vi "Read_Time_array_formation_VI.vi"(0 "Right Read MAX":string, 5 "読み取り配列":string, 9 "リード方向総合":enum16{"5’→3'", "3'→5'"}(ring), 11 "配列開始番号":i32, 12 "配列終了番号":i32) -> (1 "読み取り開始番号":i32, 3 "読み取り終了番号":i32, 4 "Base Number":i32[](array[numeric]), 6 "核酸塩基配列開始番号":i32, 10 "核酸塩基配列終了番号":i32, 13 "RRead N":i32[](array[numeric]), 14 "RR(%)":dbl, 15 "配列情報":bool[](array[boolean]))   [LabVIEW 2018]
panel:
  out "長さ 2":i32
  out "長さ":i32
  out "前":i32
  out "中心":i32
  out "後":i32
  out "部分文字列の後":string
  out "一致部分文字列":string
  out "部分文字列の前":string
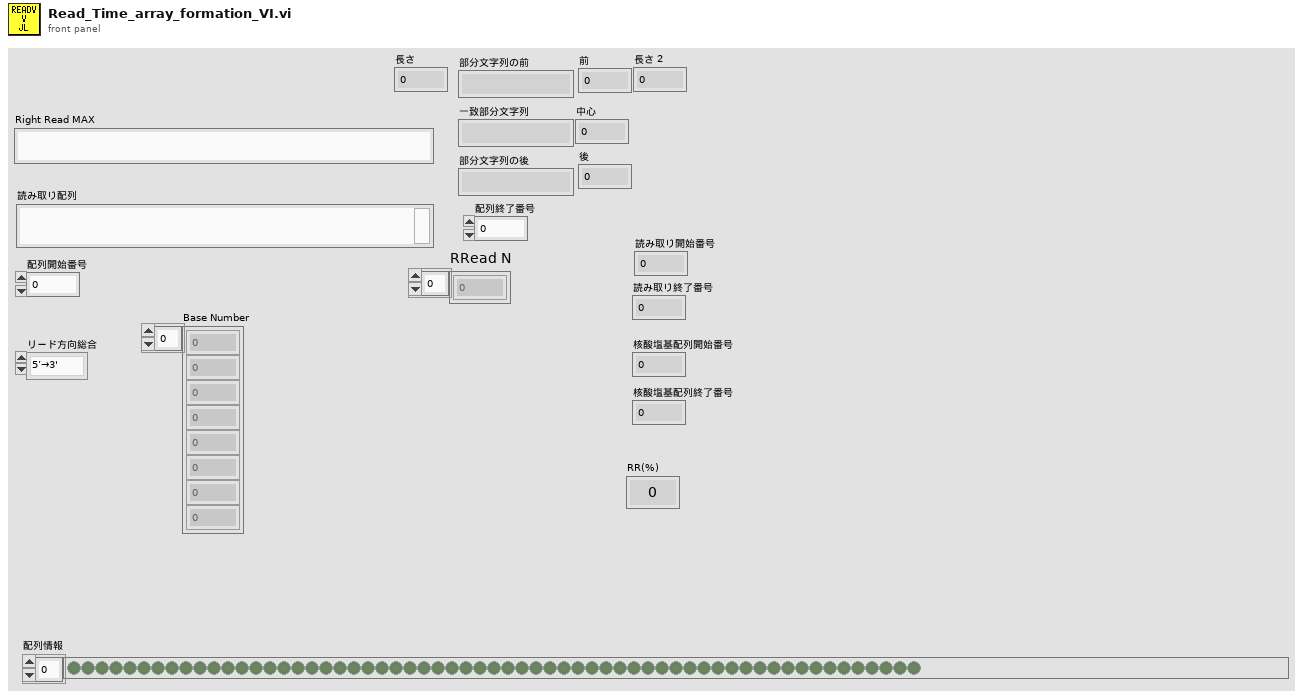
[diagram p1: front panel]
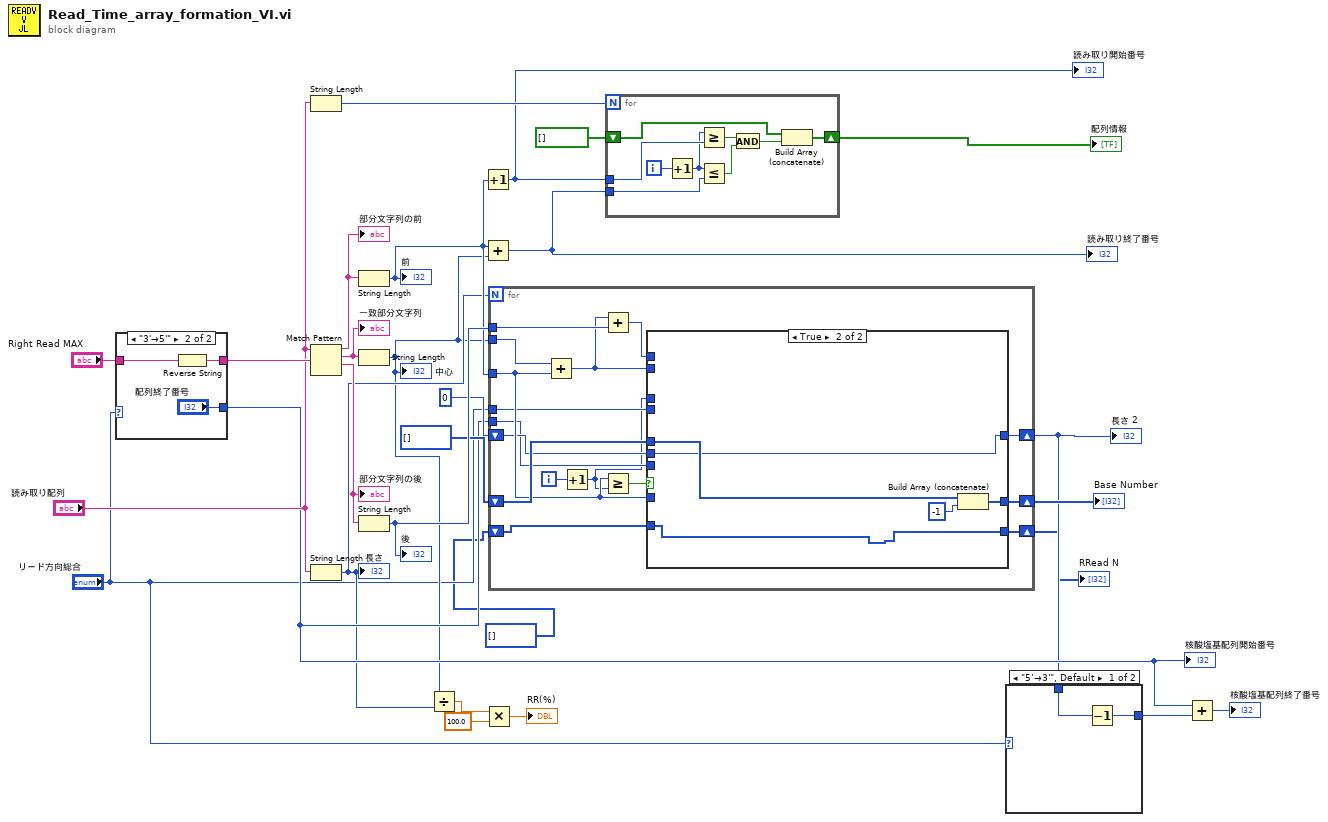
[diagram p0: block diagram]
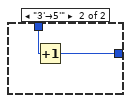
[diagram p2: hidden frame]
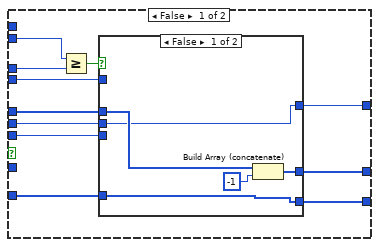
[diagram p3: hidden frame]
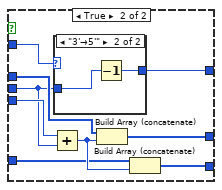
[diagram p4: hidden frame]
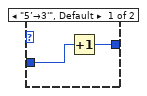
[diagram p5: hidden frame]
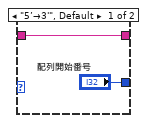
[diagram p6: hidden frame]
diagram:
  n1 = case shown="\"3'→5'\"" "リード方向総合" {
    tunnel: "Right Read MAX" -> [w30 w33]
    tunnel: [w30 w32] -> w24
    tunnel: ["配列開始番号" "配列終了番号"] -> w13
    frame "5’→3'", Default {
    }
    frame "3'→5'" {
      n2 = Reverse String(1:w33) -> (0:w32:string)
    }
  }
  "核酸塩基配列開始番号" <- w13
  n3 = String Length(string="読み取り配列") -> (length=w19:i32)
  n4 = Match Pattern(string="読み取り配列", regular expression=w24) -> (before substring=w28:string, match substring=w26:string, after substring=w27:string)  [unwired: 1 in, 1 out]
  "部分文字列の前" <- w28
  "一致部分文字列" <- w26
  "部分文字列の後" <- w27
  n5 = String Length(string="読み取り配列") -> (length=w8:i32)
  "長さ" <- w8
  n6 = String Length(string=w28) -> (length=w15:i32)
  "前" <- w15
  n7 = String Length(string=w26) -> (length=w7:i32)
  "中心" <- w7
  n8 = String Length(string=w27) -> (length=w23:i32)
  "後" <- w23
  n9 = Divide(x=w7, y=w8) -> (x/y=w6:dbl)
  n10 = Increment(x=w15) -> (x+1=w16:i32)
  "読み取り開始番号" <- w16
  n11 = Add(x=w15, y=w7) -> (x+y=w12:i32)
  "読み取り終了番号" <- w12
  n12 = Multiply(x=w6, y=100.0) -> (x*y=→"RR(%)":dbl)
  n13 = for {
    N: w8 -> [_]
    tunnel: w15 -> [w44]
    tunnel: w7 -> [w49]
    tunnel: w23 -> [w48]
    shift-right: [w46] -> w20
    shift-left: i32[] [] -> [w45]
    shift-right: [w39] -> w10
    shift-left: 0 ("長さ") -> [w40]
    tunnel: w13 -> [w38]
    tunnel: "リード方向総合" -> [w37]
    shift-right: [w35] -> w1
    shift-left: i32[] [] -> [w34]
    i -> [w41]
    n14 = Add(x=w49, y=w44) -> (x+y=w42:i32)
    n15 = Increment(x=w41) -> (x+1=w36:i32)
    n16 = Add(x=w42, y=w48) -> (x+y=w43:i32)
    n17 = Greater Or Equal?(x=w44, y=w36) -> (x >= y?=w47:bool)
    n18 = case shown="True" w47 {
      tunnel: w44 -> [_ _]
      tunnel: w42 -> [w60 _]
      tunnel: w43 -> [_ _]
      tunnel: [w54 w82] -> w46
      tunnel: w45 -> [w57 w81]
      tunnel: w36 -> [w59 _]
      tunnel: w40 -> [w56 w80]
      tunnel: [w55 w80] -> w39
      tunnel: w38 -> [w53 _]
      tunnel: w37 -> [w52 _]
      tunnel: [w51 w79] -> w35
      tunnel: w34 -> [w50 w79]
      frame False {
        n19 = Greater Or Equal?(x=w60, y=w59) -> (x >= y?=w58:bool)
        n20 = case shown="False" w58 {
          tunnel: w57 -> [w65 w73]
          tunnel: w56 -> [w62 w70]
          tunnel: [w62 w74] -> w55
          tunnel: [w64 w72] -> w54
          tunnel: w53 -> [_ w71]
          tunnel: w52 -> [_ w69]
          tunnel: [w61 w66] -> w51
          tunnel: w50 -> [w61 w67]
          frame False {
            n21 = Build Array (concatenate)(w65, -1 ("長さ")) -> (w64:i32[])
          }
          frame True {
            n22 = Add(x=w71, y=w70) -> (x+y=w68:i32)
            n23 = case shown="\"3'→5'\"" w69 {
              tunnel: [w75 w78] -> w74
              tunnel: w70 -> [w76 w77]
              frame "5’→3'", Default {
                n24 = Increment(x=w76) -> (x+1=w75:i32)
              }
              frame "3'→5'" {
                n25 = Decrement(x=w77) -> (x-1=w78:i32)
              }
            }
            n26 = Build Array (concatenate)(w73, w68) -> (w72:i32[])
            n27 = Build Array (concatenate)(w67, w68) -> (w66:i32[])
          }
        }
      }
      frame True {
        n28 = Build Array (concatenate)(w81, -1 ("長さ")) -> (w82:i32[])
      }
    }
  }
  "Base Number" <- w20
  "長さ 2" <- w10
  "RRead N" <- w1
  n29 = for {
    N: w19 -> [_]
    tunnel: w16 -> [w85]
    tunnel: w12 -> [w87]
    shift-right: [w92] -> w17
    shift-left: bool[] [] -> [w91]
    i -> [w86]
    n30 = Increment(x=w86) -> (x+1=w84:i32)
    n31 = Greater Or Equal?(x=w84, y=w85) -> (x >= y?=w90:bool)
    n32 = Less Or Equal?(x=w84, y=w87) -> (x <= y?=w88:bool)
    n33 = And(x=w90, y=w88) -> (x .and. y?=w89:bool)
    n34 = Build Array (concatenate)(w91, w89) -> (w92:bool[])
  }
  "配列情報" <- w17
  n35 = case shown="\"5’→3'\", Default" "リード方向総合" {
    tunnel: w10 -> [w94 w96]
    tunnel: [w93 w95] -> w9
    frame "5’→3'", Default {
      n36 = Decrement(x=w94) -> (x-1=w93:i32)
    }
    frame "3'→5'" {
      n37 = Increment(x=w96) -> (x+1=w95:i32)
    }
  }
  n38 = Add(x=w13, y=w9) -> (x+y=→"核酸塩基配列終了番号":i32)
